vi "Init XNET Commands Session.vi"(8 "error in (no error)":errorcluster, 11 "DUT Sample in":refnum<class "DUT Sample.lvclass">) -> (0 "error out":errorcluster, 3 "DUT Sample out":refnum<class "DUT Sample.lvclass">)   [LabVIEW 2023, in "DUT Sample.lvclass"]
uses:
  DUT Sample.lvclass
  DUT Sample.lvclass/DUT Sample.ctl
  <resource>/objmgr/xnet.rc
  <vilib>/xnet/xnet.llb/XNET Create Session (Signal Input Single-point).vi
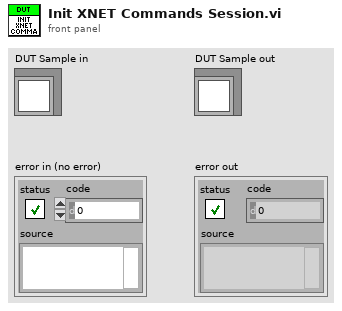
[diagram p1: front panel]
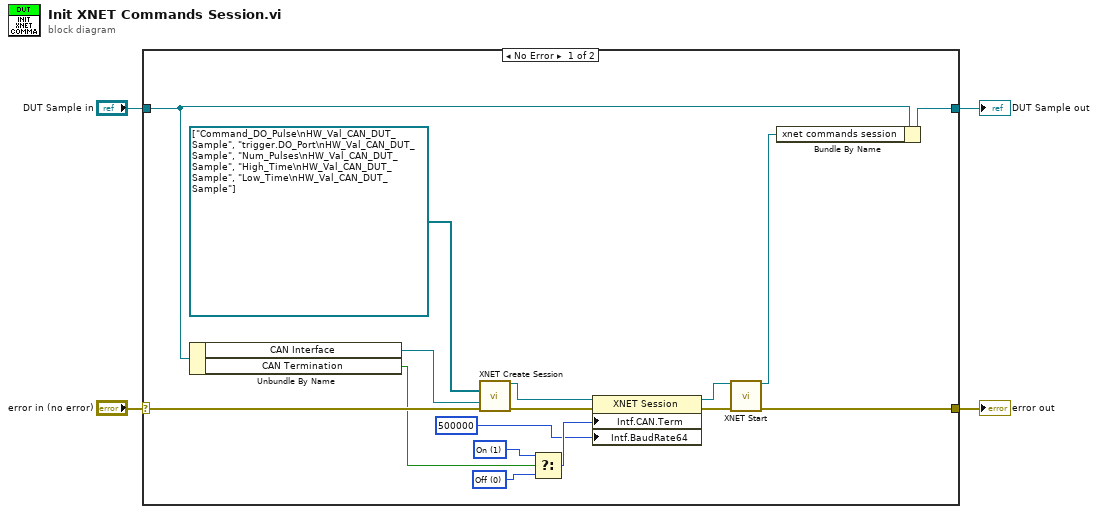
[diagram p0: block diagram]
diagram:
  n1 = case shown="No Error" "error in (no error)" {
    selector: "error in (no error)" -> [w19 w22]
    tunnel: [w18 w22] -> w3
    tunnel: [w17 w21] -> w1
    tunnel: "DUT Sample in" -> [w15 w21]
    frame No Error {
      w8 = u32 1 items=["Off", "On"] ("Interface:CAN:Termination")
      w10 = u32 0 items=["Off", "On"] ("Interface:CAN:Termination")
      n2 = Unbundle By Name(w15) -> ("CAN Interface"=w14:refnum<k21>, "CAN Termination"=w9:bool)
      n3 = call-poly <vilib>:"XNET Create Session.vi"("signal list"=refnum<k21>[] ["Command_DO_Pulse\nHW_Val_CAN_DUT_Sample", "trigger.DO_Port\nHW_Val_CAN_DUT_Sample", "Num_Pulses\nHW_Val_CAN_DUT_Sample", "High_Time\nHW_Val_CAN_DUT_Sample", "Low_Time\nHW_Val_CAN_DUT_Sample"] ("Select Signal List from database"), "interface"=w14, "error in (no error)"=w19) -> ("session out"=w12:refnum<k21>, "error out"=w20:errorcluster)  [unwired: 11 out]
      n4 = Select(t=w8, s=w9, f=w10) -> (s? t:f=w7:u32)
      n5 = property class="XNET Session"(reference=w12, error in=w20, "Intf.CAN.Term"=w7, "Intf.BaudRate64"=u64 500000 ("Interface:64bit Baud Rate")) -> (reference out=w11:refnum<k21>, error out=w13:errorcluster)
      n6 = call <vilib>:"XNET Start.vi"("session in"=w11, "error in (no error)"=w13) -> ("session out"=w16:refnum<k21>, "error out"=w18:errorcluster)  [unwired: 12 in]
      n7 = Bundle By Name(cluster=w15, "xnet commands session"=w16) -> (w17:refnum<class "DUT Sample.lvclass">)
    }
    frame Error {
    }
  }
  "error out" <- w3
  "DUT Sample out" <- w1
